vi "R_ID_index_arr.vi"(8 "error in (no error)":errorcluster caption="错误输入（无错误）", 11 "Procotol_class输入":refnum<class "Procotol_class.lvclass">) -> (0 "error out":errorcluster caption="错误输出", 2 "ID_index_arr":i32[][](array[numeric]), 3 "Procotol_class输出":refnum<class "Procotol_class.lvclass">)   [LabVIEW 2025, in "Procotol_class.lvclass"]
uses:
  Procotol_class.lvclass
  Procotol_class.lvclass/Procotol_class.ctl
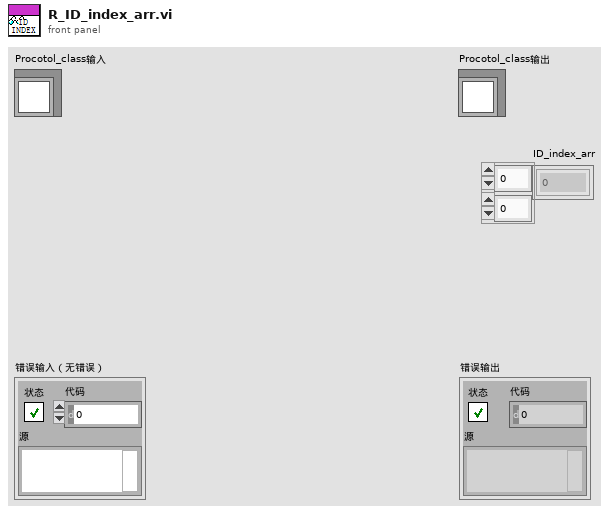
[diagram p1: front panel]
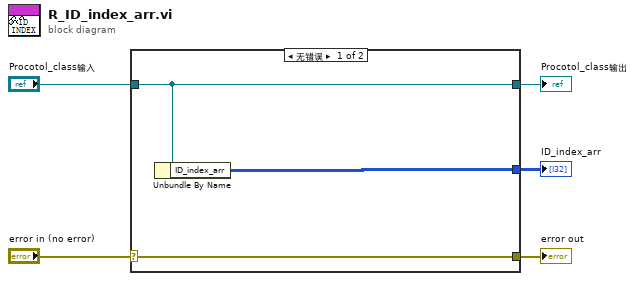
[diagram p0: block diagram]
diagram:
  n1 = case shown="无错误" "error in (no error)" {
    selector: "error in (no error)" -> [w8 w9]
    tunnel: [w8 w9] -> w4
    tunnel: [w7 w10] -> w2
    tunnel: "Procotol_class输入" -> [w7 w10]
    tunnel: [w6 _] -> w1
    frame No Error {
      n2 = Unbundle By Name(w7) -> ("ID_index_arr"=w6:i32[][])
    }
    frame Error {
    }
  }
  "error out" <- w4
  "Procotol_class输出" <- w2
  "ID_index_arr" <- w1
